vi "Create SimpleText Paragraph.vi"(8 "error in (no error)":errorcluster, 10 "simpleText":string, 11 "ooWriter in":refnum<class "ooWriter.lvclass">) -> (0 "error out":errorcluster, 2 "SimpleTextParagraph":refnum<k24>, 3 "ooWriter out":refnum<class "ooWriter.lvclass">)   [LabVIEW 2009, in "ooWriter.lvclass"]
uses:
  ooWriter.lvclass
  C:/Projets/LAVAG/OpenOfficeRGT/AODL/DLLs/AODL.dll
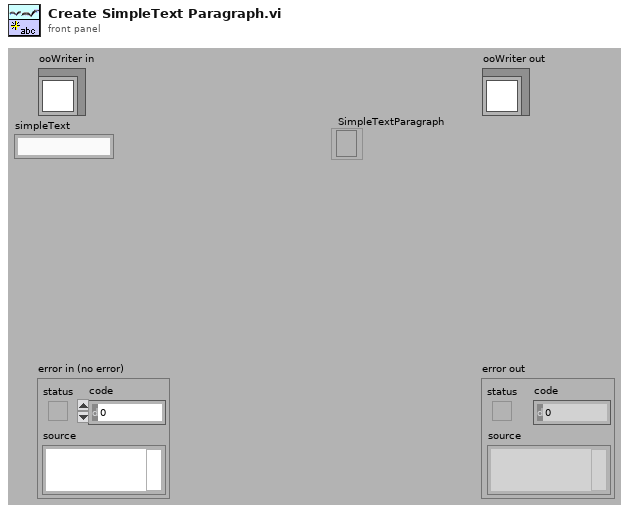
[diagram p1: front panel]
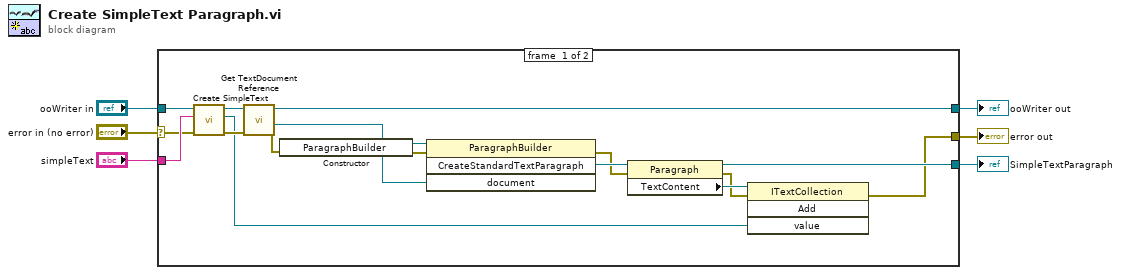
[diagram p0: block diagram]
diagram:
  n1 = case shown="No Error" "error in (no error)" {
    selector: "error in (no error)" -> [w9 w25]
    tunnel: [w13 w25] -> w5
    tunnel: [w17 w24] -> w3
    tunnel: "ooWriter in" -> [w11 w24]
    tunnel: "simpleText" -> [w12 _]
    tunnel: [w19 _] -> w1
    frame #0 {
      n2 = call-dynamic "Create SimpleText.vi"("error in (no error)"=w9, "simpleText"=w12, "ooDocument"=w11) -> ("error out"=w8:errorcluster, "SimpleText"=w7:refnum<k24>, "ooDocument out"=w10:refnum<class "ooWriter.lvclass">)  [unwired: 6 in]
      n3 = call-dynamic "Get TextDocument Reference.vi"("error in (no error)"=w8, "ooWriter in"=w10) -> ("error out"=w16:errorcluster, "Document"=w18:refnum<k24>, "ooWriter out"=w17:refnum<class "ooWriter.lvclass">)  [unwired: 7 in]
      n4 = constructor class="ParagraphBuilder"(error in=w16) -> (reference out=w22:refnum<k24>, error out=w23:errorcluster)  [unwired: 2 in, 1 out]
      n5 = invoke class="ParagraphBuilder" method="CreateStandardTextParagraph"(reference=w22, error in=w23, "document"=w18) -> (error out=w15:errorcluster, "CreateStandardTextParagraph"=w21:refnum<k24>)  [unwired: 1 in, 2 out]
      n6 = property class="Paragraph"(reference=w21, error in=w15) -> (reference out=w19:refnum<k24>, error out=w14:errorcluster, "TextContent"=w20:refnum<k24>)
      n7 = invoke class="ITextCollection" method="Add"(reference=w20, error in=w14, "value"=w7) -> (error out=w13:errorcluster)  [unwired: 1 in, 3 out]
    }
    frame #1 {
    }
  }
  "error out" <- w5
  "ooWriter out" <- w3
  "SimpleTextParagraph" <- w1
